vi "Native_GetStringConstantValue.vi"() -> ()   [LabVIEW 2024]
panel:
  out "error out":errorcluster caption="错误输出"
  out "value":variant
  in  "constant_id":u32
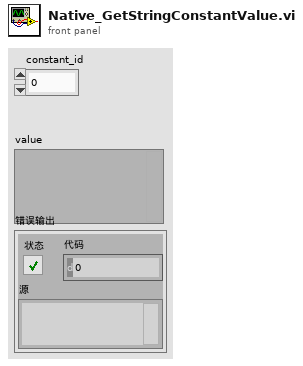
[diagram p1: front panel]
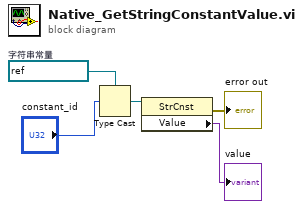
[diagram p0: block diagram]
diagram:
  w4 = refnum<vi> refnum  # 字符串常量
  n1 = Type Cast ("强制类型转换")(type=w4, x="constant_id") -> (*(type *) &x=w3:refnum<vi>)
  n2 = property on="属性节点" class="StrCnst"(reference=w3) -> (error out=→"error out":errorcluster, "Value"=→"value":variant)  [unwired: 1 in, 1 out]
